vi "VHistFile - Save newest App histories.vi"(6 "file params":T2={"path pattern"=enum."Y\\M\\D\\Tag.ext", "file extension (.bin)"=".bin"}, 8 "error in":errorcluster, 9 "log directory":path=path "DataLog", 11 "app vc handles":T1[](array[typedef])) -> (0 "error out":errorcluster)   [LabVIEW 2021]
doc: "The VI acquires the newest history data for all variables in the specified variable contexts that have an alias associated. Then VI writes the history data of each variable to the respective log file(s); herewith, VI uses an alias associated with the variable as a <b>file tag</b>. If an array of context handles is empty, VI saves the newest histories for all variables that have alias associated. The VI automatically recognizes variable datatypes and saves data values in appropriate formats. If a variable has a datatype that the VI does not support, it saves variable values in the Flattened-To-String format.\n\n::: CalcExpress Toolkit :::\nCopyright (c) 2000-2026 Konstantin Shifershteyn. All rights reserved."
uses:
  cetypes.llb/VarMan Variable Context Handle.ctl
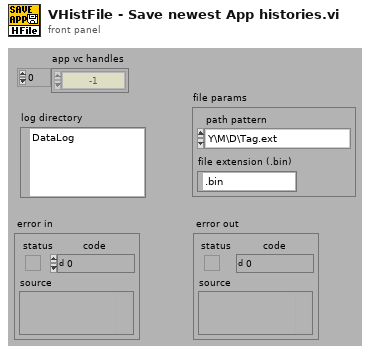
[diagram p1: front panel]
types:
  T1 = typedef "VarMan Variable Context Handle.ctl" = i32
  T2 = cluster{"path pattern":enum32{"Y\\M\\D\\Tag.ext", "Y\\M\\D\\Tag [Y-M-D].ext", "Y-M-D\\Tag.ext", "Y-M-D\\Tag [Y-M-D].ext", "Tag [Y-M-D].ext"}, "file extension (.bin)":string}
  T3 = typedef "VarMan Alias Info Cluster.ctl" = cluster{"alias":string, "vc handle":T1, "var name":string, "type":u32, "history":bool}
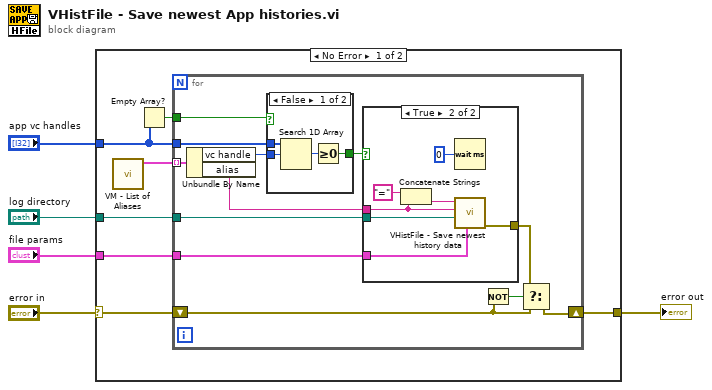
[diagram p0: block diagram]
diagram:
  n1 = case shown="No Error" "error in" {
    selector: "error in" -> [w6 w37]
    tunnel: "log directory" -> [w12 _]
    tunnel: [w10 w37] -> w4
    tunnel: "app vc handles" -> [w8 _]
    tunnel: "file params" -> [w7 _]
    frame No Error {
      n2 = call "VM - List of Aliases.vi"() -> ("aliases info"=w11:T3[])  [unwired: 10 in, 1 out]
      n3 = Empty Array?(array=w8) -> (empty?=w9:bool)
      n4 = for {
        tunnel: w11 -> [w23] mode=indexing
        tunnel: w12 -> [w22]
        shift-right: [w19] -> w10
        shift-left: w6 -> [w13]
        tunnel: w8 -> [w17]
        tunnel: w9 -> [w16]
        tunnel: w7 -> [w14]
        n5 = Unbundle By Name(w23) -> ("vc handle"=w18:T1, "alias"=w24:string)
        n6 = case shown="False" w16 {
          selector: w16 -> [_ w29]
          tunnel: w18 -> [w28 _]
          tunnel: w17 -> [w27 _]
          tunnel: [w25 w29] -> w15
          frame False {
            n7 = Search 1D Array(1D array=w27, element=w28) -> (index of element=w26:i32)  [unwired: 1 in]
            n8 = Greater Or Equal To 0?(x=w26) -> (x >= 0?=w25:bool)
          }
          frame True {
          }
        }
        n9 = case shown="True" w15 {
          tunnel: w24 -> [_ w34]
          tunnel: w22 -> [_ w33]
          tunnel: [_ w32] -> w20
          tunnel: w14 -> [_ w30]
          frame False {
          }
          frame True {
            n10 = Concatenate Strings("=", w34) -> (w35:string)
            n11 = Wait (ms)(milliseconds to wait=u32 0) -> ()  [unwired: 1 out]
            n12 = call "VHistFile - Save newest history data.vi"("file params"=w30, "log directory"=w33, "file tag"=w34, "name_spec"=w35) -> ("error out"=w32:errorcluster)  [unwired: 4 in, 3 out]
          }
        }
        n13 = Not(x=w13) -> (.not. x?=w21:bool)
        n14 = Select(t=w20, s=w21, f=w13) -> (s? t:f=w19:errorcluster)
      }
    }
    frame Error {
    }
  }
  "error out" <- w4
